vi "EmulationSandboxKeyboard.vi"() -> ()   [LabVIEW 2026]
uses:
  KeyboardAndMouseDataAcquisition.ctl
  replay/KeyboardReplayKey.ctl
  KeyType.ctl
  <vilib>/Wovalab/Utilities/Helper Loop Periodic Timing/Helper Loop Periodic Timing.lvclass/Helper Loop Periodic Timing.ctl
  MouseLUTSelector.ctl
  aee89bbf-916d-4481-9317-930c4b9b316a.vi
  be5614b6-9380-4e19-a85a-dfb08a87b78c.vi
  <vilib>/Wovalab/Utilities/Helper Loop Periodic Timing/Read Current Number Of Execution.vi
  <vilib>/Wovalab/Utilities/Helper Loop Periodic Timing/Stop Helper Loop Internal.vi
  <vilib>/Wovalab/Utilities/Helper Loop Periodic Timing/U32 Max Value--constant.vi
  <vilib>/Wovalab/Utilities/Helper Loop Periodic Timing/Update Last Execution Time.vi
  <vilib>/Wovalab/Utilities/Helper Loop Periodic Timing/Loops Events AE.vi
  <vilib>/Wovalab/Utilities/Helper Loop Periodic Timing/Notify Monitoring Window.vi
  <vilib>/Wovalab/Utilities/Helper Loop Periodic Timing/Monitoring--global.vi
  <userlib>/_OpenG.lib/comparison/comparison.llb/U8 Changed__ogtk.vi
  <vilib>/Wovalab/Utilities/Helper Loop Periodic Timing/Late Execution Mode--enum.ctl
  <vilib>/Wovalab/Utilities/Helper Loop Periodic Timing/Helper Loop Periodic Timing.lvclass
  replay/Replay/src/Libraries/Replay/Replay.lvlib
  <userlib>/_OpenG.lib/comparison/comparison.llb/openg_comparison__ogtk.lvlib
  a2901e3a-1446-44b0-a1b1-14ac9caae76d.vi
  User32.dll
panel:
  out "Array 4":T1(array[cluster])
  out "Array 2":T2(array[cluster])
  out "Array":T3(array[ring])
  out "Unimplemented":bool
  out "Boolean":bool
  out "error out":errorcluster
  out "ReplaySamples":T4[](array[typedef])
  in  "Run ID":string
  out "Virtual Key 2":T5=164
  in  "keyType Recorded":T6=enum."1"
  out "Virtual Key":T5=164
  out "Key":T7(ring)
  in  "Exit":bool
  in  "Stop":bool
  in  "Start":bool
  out "Keyboard Keys Pressed":T3(array[ring])
  out "Array 3":T4[](array[typedef])
  # "wqeeeeeeeeeeeeeeeeeeeeeeeeeeeeeeeeeeeeeeeeeeeeeeeeeeeeeeeeeeeeeeeeeeeeeeeeeeeeee"
  # "sssssssssssssddddddddddddddddddddddddddddddddddddddddddd"
  # "fsdsdsdsdsdsdsdsdsdsdaaaaaaaaaaaaaaaaaaaaaaaaaaaaaaaaa"
  # "qweeeeeeeeewqqqqqqqqqqqqqqqqqqqqqqqqqqqqqqqqqqqqqqqqqq"
  # "sdffffffffffffffffffAAAAAA"
  # "sdsdsdsdsdsdsdsdsdsdaaaaaaaaaaaaaaaaaaaaaaaaaaaaaaaaaaaaaaaaaaaaaaaaaaaaaaaaaaa"
  # "rewwwwwwwwwwwwwwwwwwwwrewwerrrrrrrrrewwwwwwwwwwwwww"
  # "rew"
  # "rrrrrrrrreeeeeeeewwwwwwwwww"
  # "rrrrrrrreeeeeeeeeeewwwwwwwwwwwwwww"
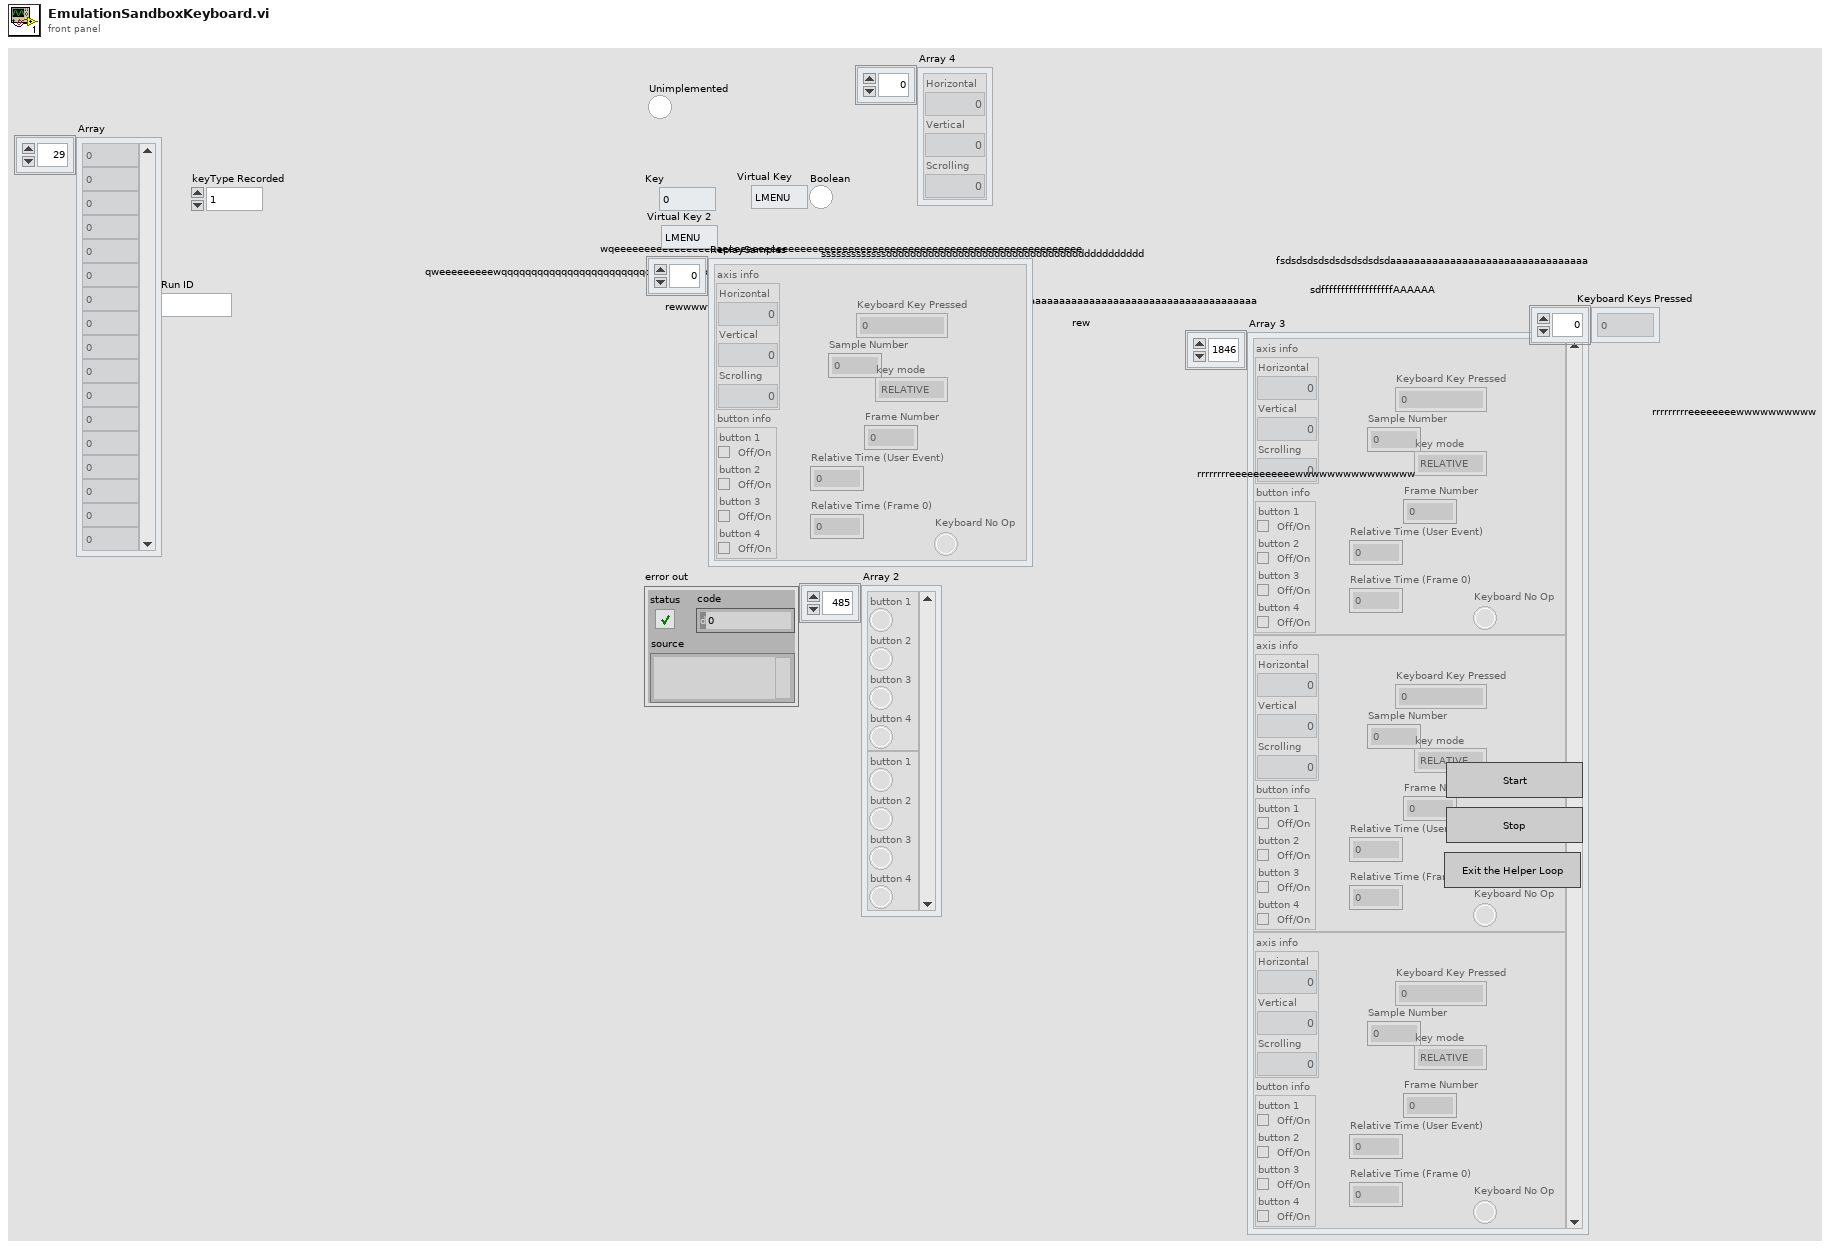
[diagram p1: front panel]
types:
  T1 = cluster{"Horizontal":i32, "Vertical":i32, "Scrolling":i32}[]
  T2 = cluster{"button 1":bool, "button 2":bool, "button 3":bool, "button 4":bool}[]
  T3 = enum16{"0", "1", "2", "3", "4", "5", "6", "7", "8", "9", "A", "B", "C", "D", "E", "F", "G", "H", "I", "J", "K", "L", "M", "N", "O", "P", "Q", "R", "S", "T", "U", "V", "W", "X", "Y", "Z", "F1", "F2", "F3", "F4", "F5", "F6", "F7", "F8", "F9", "F10", "F11", "F12", "F13", "F14", "F15", "ADD", "BACK", "BACKSLASH", "CAPITAL", "COMMA", "DECIMAL", "DELETE", "DIVIDE", "DOWN", "END", "EQUALS", "ESCAPE", "GRAVE (`)", "HOME", "INSERT", "LBRACKET", "LCONTROL", "LEFT", "L ALT", "LSHIFT", "LWIN", "MINUS", "MULTIPLY", "NEXT", "NUMLOCK", "NUMPAD_0", "NUMPAD_1", "NUMPAD_2", "NUMPAD_3", "NUMPAD_4", "NUMPAD_5", "NUMPAD_6", "NUMPAD_7", "NUMPAD_8", "NUMPAD_9", "PAUSE", "PERIOD", "PRIOR (PG UP)", "RBRACKET", "RCONTROL", "RETURN", "RIGHT", "R ALT", "RSHIFT", "RWIN", "SCROLL", "SEMICOLON", "SLASH", "SPACE", "SUBTRACT", "TAB", "UP", "ENTER (num pad)", "' (quote)"}[]
  T4 = typedef "KeyboardAndMouseDataAcquisition.ctl" = cluster{"axis info":cluster{"Horizontal":i32, "Vertical":i32, "Scrolling":i32}, "button info":cluster{"button 1":bool, "button 2":bool, "button 3":bool, "button 4":bool}, "Relative Time (User Event)":dbl, "Sample Number":u32, "Relative Time (Frame 0)":dbl, "key mode":enum16{"RELATIVE", "ABSOLUTE"}, "Frame Number":u32, "Keyboard Key Pressed":enum16{"0", "1", "2", "3", "4", "5", "6", "7", "8", "9", "A", "B", "C", "D", "E", "F", "G", "H", "I", "J", "K", "L", "M", "N", "O", "P", "Q", "R", "S", "T", "U", "V", "W", "X", "Y", "Z", "F1", "F2", "F3", "F4", "F5", "F6", "F7", "F8", "F9", "F10", "F11", "F12", "F13", "F14", "F15", "ADD", "BACK", "BACKSLASH", "CAPITAL", "COMMA", "DECIMAL", "DELETE", "DIVIDE", "DOWN", "END", "EQUALS", "ESCAPE", "GRAVE (`)", "HOME", "INSERT", "LBRACKET", "LCONTROL", "LEFT", "L ALT", "LSHIFT", "LWIN", "MINUS", "MULTIPLY", "NEXT", "NUMLOCK", "NUMPAD_0", "NUMPAD_1", "NUMPAD_2", "NUMPAD_3", "NUMPAD_4", "NUMPAD_5", "NUMPAD_6", "NUMPAD_7", "NUMPAD_8", "NUMPAD_9", "PAUSE", "PERIOD", "PRIOR (PG UP)", "RBRACKET", "RCONTROL", "RETURN", "RIGHT", "R ALT", "RSHIFT", "RWIN", "SCROLL", "SEMICOLON", "SLASH", "SPACE", "SUBTRACT", "TAB", "UP", "ENTER (num pad)", "' (quote)"}, "Keyboard No Op":bool}
  T5 = typedef "KeyboardReplayKey.ctl" = u8
  T6 = typedef "KeyType.ctl" = enum16{"0", "1", "2", "3", "4", "5", "6", "7", "8", "9", "A", "B", "C", "D", "E", "F", "G", "H", "I", "J", "K", "L", "M", "N", "O", "P", "Q", "R", "S", "T", "U", "V", "W", "X", "Y", "Z", "F1", "F2", "F3", "F4", "F5", "F6", "F7", "F8", "F9", "F10", "F11", "F12", "F13", "F14", "F15", "ADD", "BACK", "BACKSLASH", "CAPITAL", "COMMA", "DECIMAL", "DELETE", "DIVIDE", "DOWN", "END", "EQUALS", "ESCAPE", "GRAVE (`)", "HOME", "INSERT", "LBRACKET", "LCONTROL", "LEFT", "L ALT", "LSHIFT", "LWIN", "MINUS", "MULTIPLY", "NEXT", "NUMLOCK", "NUMPAD_0", "NUMPAD_1", "NUMPAD_2", "NUMPAD_3", "NUMPAD_4", "NUMPAD_5", "NUMPAD_6", "NUMPAD_7", "NUMPAD_8", "NUMPAD_9", "PAUSE", "PERIOD", "PRIOR (PG UP)", "RBRACKET", "RCONTROL", "RETURN", "RIGHT", "R ALT", "RSHIFT", "RWIN", "SCROLL", "SEMICOLON", "SLASH", "SPACE", "SUBTRACT", "TAB", "UP", "ENTER (num pad)", "' (quote)"}
  T7 = enum16{"0", "1", "2", "3", "4", "5", "6", "7", "8", "9", "A", "B", "C", "D", "E", "F", "G", "H", "I", "J", "K", "L", "M", "N", "O", "P", "Q", "R", "S", "T", "U", "V", "W", "X", "Y", "Z", "F1", "F2", "F3", "F4", "F5", "F6", "F7", "F8", "F9", "F10", "F11", "F12", "F13", "F14", "F15", "ADD", "BACK", "BACKSLASH", "CAPITAL", "COMMA", "DECIMAL", "DELETE", "DIVIDE", "DOWN", "END", "EQUALS", "ESCAPE", "GRAVE (`)", "HOME", "INSERT", "LBRACKET", "LCONTROL", "LEFT", "L ALT", "LSHIFT", "LWIN", "MINUS", "MULTIPLY", "NEXT", "NUMLOCK", "NUMPAD_0", "NUMPAD_1", "NUMPAD_2", "NUMPAD_3", "NUMPAD_4", "NUMPAD_5", "NUMPAD_6", "NUMPAD_7", "NUMPAD_8", "NUMPAD_9", "PAUSE", "PERIOD", "PRIOR (PG UP)", "RBRACKET", "RCONTROL", "RETURN", "RIGHT", "R ALT", "RSHIFT", "RWIN", "SCROLL", "SEMICOLON", "SLASH", "SPACE", "SUBTRACT", "TAB", "UP", "ENTER (num pad)", "' (quote)"}
  T8 = typedef "Wovalab_lib_Utilities.lvlib/Helper Loop Periodic Timing.lvclass/Late Execution Mode--enum.ctl" = enum16{"No change", "Process missed periods ignoring original phase", "Process missed periods maintaining original phase"}
  T9 = typedef "MouseLUTSelector.ctl" = enum16{"Initialize", "Get Button and Axis Info", "Assign Button and Axis Info to Sample Number"}
  T10 = typedef "SerializedKeyPress.ctl" = cluster{"Key Down":bool, "Key Up":bool, "Key":enum16{"0", "1", "2", "3", "4", "5", "6", "7", "8", "9", "A", "B", "C", "D", "E", "F", "G", "H", "I", "J", "K", "L", "M", "N", "O", "P", "Q", "R", "S", "T", "U", "V", "W", "X", "Y", "Z", "F1", "F2", "F3", "F4", "F5", "F6", "F7", "F8", "F9", "F10", "F11", "F12", "F13", "F14", "F15", "ADD", "BACK", "BACKSLASH", "CAPITAL", "COMMA", "DECIMAL", "DELETE", "DIVIDE", "DOWN", "END", "EQUALS", "ESCAPE", "GRAVE (`)", "HOME", "INSERT", "LBRACKET", "LCONTROL", "LEFT", "L ALT", "LSHIFT", "LWIN", "MINUS", "MULTIPLY", "NEXT", "NUMLOCK", "NUMPAD_0", "NUMPAD_1", "NUMPAD_2", "NUMPAD_3", "NUMPAD_4", "NUMPAD_5", "NUMPAD_6", "NUMPAD_7", "NUMPAD_8", "NUMPAD_9", "PAUSE", "PERIOD", "PRIOR (PG UP)", "RBRACKET", "RCONTROL", "RETURN", "RIGHT", "R ALT", "RSHIFT", "RWIN", "SCROLL", "SEMICOLON", "SLASH", "SPACE", "SUBTRACT", "TAB", "UP", "ENTER (num pad)", "' (quote)"}}
  T11 = cluster{"Horizontal":i32, "Vertical":i32, "Scrolling":i32}
  T12 = cluster{"button 1":bool, "button 2":bool, "button 3":bool, "button 4":bool}
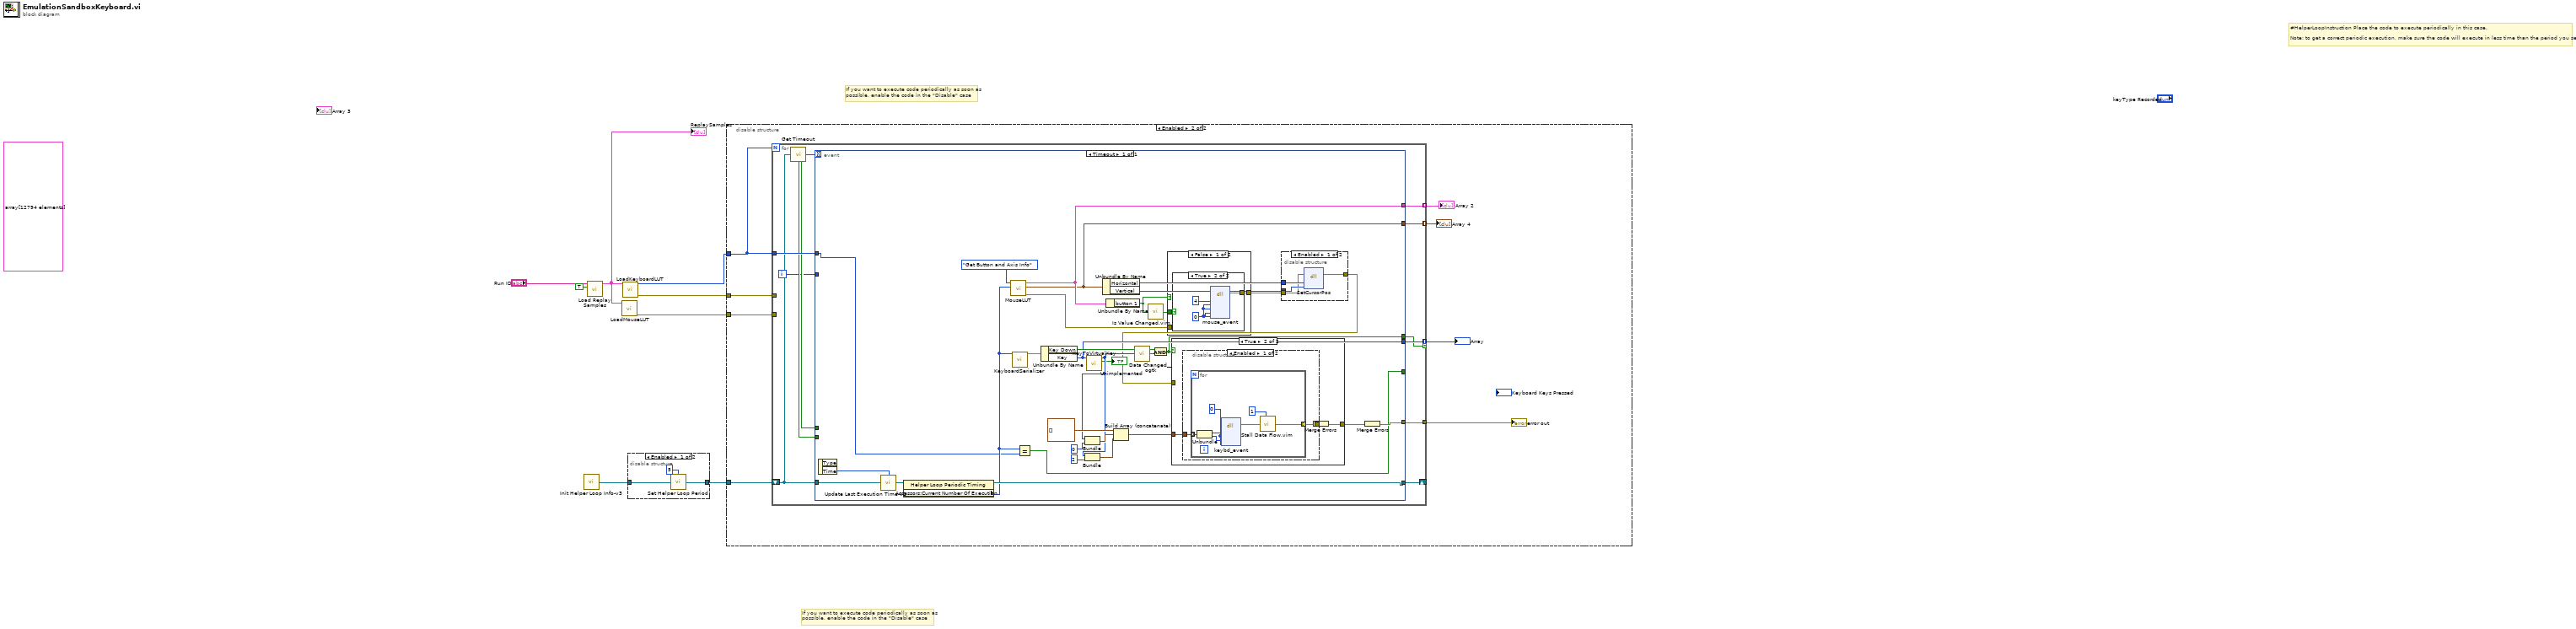
[diagram p0: block diagram]
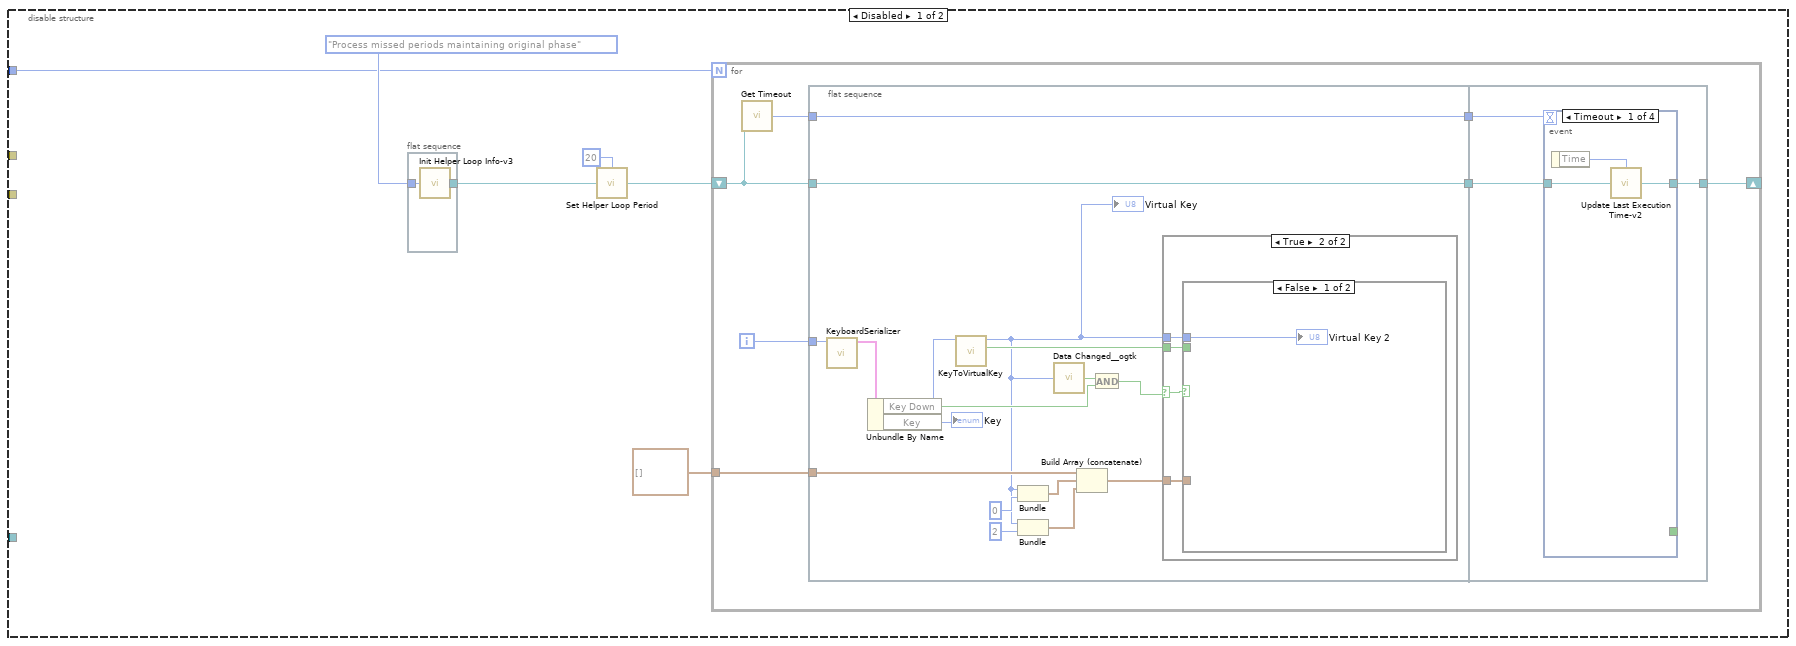
[diagram p3: hidden frame]
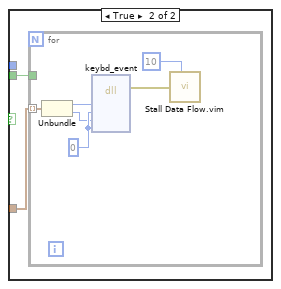
[diagram p5: hidden frame]
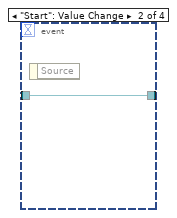
[diagram p6: hidden frame]
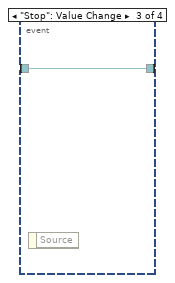
[diagram p7: hidden frame]
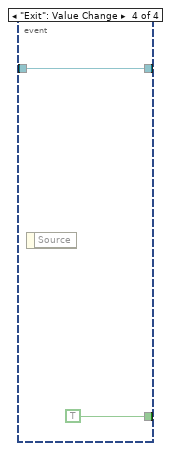
[diagram p8: hidden frame]
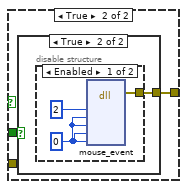
[diagram p11: hidden frame]
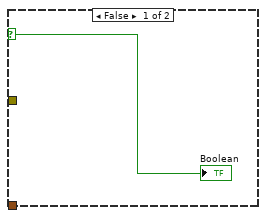
[diagram p14: hidden frame]
diagram:
  (unwired) T4[] array[12794 elements] ("Array 3")
  # "If you want to execute code periodically as soon as possible, enable the code in the \"Disable\" case"
  # "If you want to execute code periodically as soon as possible, enable the code in the \"Disable\" case"
  # "#HelperLoopInstruction Place the code to execute periodically in this case.\n\nNote: to get a correct periodic execution, make sure the code will execute in less time than the period you set."
  n1 = call <vilib>:"Init Helper Loop Info-v3.vi"() -> ("Helper Loop Periodic Timing"=w4:refnum<class "Helper Loop Periodic Timing.lvclass">)  [unwired: 2 in]
  n2 = call "Load Replay Samples.vi"("Load From ProgramData"=TRUE, "Run ID"="Run ID") -> ("ReplaySamples"=w2:T4[])  [unwired: 8 in, 1 out]
  "ReplaySamples" <- w2
  n3 = call "LoadMouseLUT.vi"("Metadata"=w2) -> ("error out"=w1:errorcluster)  [unwired: 10 in]
  n4 = call "LoadKeyboardLUT.vi"("Metadata"=w2) -> ("error out"=w6:errorcluster, "Samples"=w5:u32)  [unwired: 9 in]
  n5 = disable-structure shown="Enabled" {
    disable-tunnel: w4 -> [w11 w12]
    disable-tunnel: [w10 w12] -> w3
    frame Enabled {
      n6 = call <vilib>:"Set Helper Loop Period.vi"("Period (ms)"=5, "Helper Loop Periodic Timing in"=w11) -> ("Helper Loop Periodic Timing out"=w10:refnum<class "Helper Loop Periodic Timing.lvclass">)  [unwired: 13 in]
    }
    frame Disabled {
    }
  }
  n7 = disable-structure shown="Enabled" {
    disable-tunnel: w5 -> [w13 w75]
    disable-tunnel: w6 -> [_ w76]
    disable-tunnel: w3 -> [_ w74]
    disable-tunnel: w1 -> [_ w73]
    frame Disabled {
      n8 = flat-sequence {
        tunnel: [w69] -> w17
        tunnel: Late_Execution_Mode--enum."Process missed periods maintaining original phase" ("Late Execution Mode (Process missed periods ignoring original phase)") -> [w68]
        frame #0 {
          n9 = call <vilib>:"Init Helper Loop Info-v3.vi"("Late Execution Mode (Process missed periods ignoring original phase)"=w68) -> ("Helper Loop Periodic Timing"=w69:refnum<class "Helper Loop Periodic Timing.lvclass">)  [unwired: 1 in]
        }
      }
      n10 = call <vilib>:"Set Helper Loop Period.vi"("Period (ms)"=20, "Helper Loop Periodic Timing in"=w17) -> ("Helper Loop Periodic Timing out"=w18:refnum<class "Helper Loop Periodic Timing.lvclass">)  [unwired: 13 in]
      n11 = for {
        N: w13 -> [_]
        shift-right: [w23] -> _
        shift-left: w18 -> [w24]
        tunnel: cluster{i32, i32}[] [] -> [w20]
        i -> [w19]
        n12 = call <vilib>:"Get Timeout.vi"("Helper Loop Periodic Timing"=w24) -> ("Timeout (ms)"=w25:i32)  [unwired: 12 in, 2 out]
        n13 = flat-sequence {
          tunnel: w24 -> [w40]
          tunnel: w25 -> [w41]
          tunnel: [w41] -> w22
          tunnel: [w40] -> w21
          tunnel: w20 -> [w35]
          tunnel: w19 -> [w29]
          tunnel: [w55] -> w23
          tunnel: w22 -> [w57]
          tunnel: w21 -> [w56]
          frame #0 {
            n14 = call "KeyboardSerializer.vi"("Sample Number"=w29) -> ("SerializedKeyPress"=w28:T10)  [unwired: 9 in, 1 out]
            n15 = Unbundle By Name(w28) -> ("Key Down"=w31:bool, "Key"=w39:T7)
            "Key" <- w39
            n16 = call "KeyToVirtualKey.vi"("keyType Recorded"=w39) -> ("Unimplemented"=w27:bool, "Virtual Key"=w26:T5)  [unwired: 9 in]
            "Virtual Key" <- w26
            n17 = Bundle("Virtual Key"=w26, 0) -> (w37:cluster{"Virtual Key":T5, i32})  [unwired: 1 in]
            n18 = Bundle("Virtual Key"=w26, 2) -> (w38:cluster{"Virtual Key":T5, i32})  [unwired: 1 in]
            n19 = call-poly <userlib>:"Data Changed__ogtk.vi"("U8"=w26) -> ("Changed"=w32:bool)
            n20 = Build Array (concatenate)(w35, w37, w38) -> (w33:cluster{"Virtual Key":i32, i32}[])
            n21 = And(x=w32, y=w31) -> (x .and. y?=w30:bool)
            n22 = case shown="True" w30 {
              selector: w30 -> [_ w43]
              tunnel: w33 -> [_ w45]
              tunnel: w27 -> [_ w44]
              tunnel: w26 -> [_ w42]
              frame False {
              }
              frame True {
                n23 = case shown="False" w43 {
                  tunnel: w45 -> [_ w48]
                  tunnel: w44 -> [_ w47]
                  tunnel: w42 -> [w46 _]
                  frame False {
                    "Virtual Key 2" <- w46
                  }
                  frame True {
                    n24 = for {
                      tunnel: w48 -> [w53] mode=indexing
                      tunnel: w47 -> [_]
                      w54 = u32 0 ("dwFlags")
                      n25 = Unbundle(w53) -> ("Virtual Key"=w52:i32, w51:i32)
                      n26 = dll-call lib="user32.dll" fn="keybd_event"("bVk"=w52, "bScan"=w54, "dwFlags"=w51, "dwExtraInfo"=w54) -> (error out=w50:errorcluster)  [unwired: 8 in, 1 out]
                      n27 = call "Stall Data Flow.vim"("value in"=w50, "milliseconds to wait"=u32 10) -> ()  [unwired: 2 out]
                    }
                  }
                }
              }
            }
          }
          frame #1 {
            n28 = event shown="[0] Timeout" {
              selector: _ -> [_ _ _ _]
              dyn-events: _ -> [_ _ _ _]
              timeout: w57 -> [_ _ _ _]
              tunnel: w56 -> [w60 w63 w65 w67]
              tunnel: [w59 w62 w64 w67] -> w55
              tunnel: [_ _ _ TRUE] -> _
              event Timeout {
                n29 = event-data() -> ("Time"=w58:u32)  [unwired: 1 in]
                n30 = call <vilib>:"Update Last Execution Time-v2.vi"("Time"=w58, "Helper Loop Periodic Timing in"=w60) -> ("Helper Loop Periodic Timing out"=w59:refnum<class "Helper Loop Periodic Timing.lvclass">)  [unwired: 12 in, 1 out]
              }
              event "Start": Value Change {
                # "#HelperLoopInstruction Set the desired period (in ms), here."
                n31 = call <vilib>:"Set Helper Loop Period.vi"("Period (ms)"=500, "Helper Loop Periodic Timing in"=w63) -> ("Helper Loop Periodic Timing out"=w62:refnum<class "Helper Loop Periodic Timing.lvclass">)  [unwired: 13 in]
                n32 = event-data() -> ()  [unwired: 1 in, 1 out]
              }
              event "Stop": Value Change {
                n33 = call <vilib>:"Stop Helper Loop.vi"("Helper Loop Periodic Timing in"=w65) -> ("Helper Loop Periodic Timing out"=w64:refnum<class "Helper Loop Periodic Timing.lvclass">)
                n34 = event-data() -> ()  [unwired: 1 in, 1 out]
              }
              event "Exit": Value Change {
                n35 = event-data() -> ()  [unwired: 1 in, 1 out]
              }
            }
          }
        }
      }
    }
    frame Enabled {
      n36 = for {
        N: w75 -> [_]
        tunnel: [w89] -> w77
        tunnel: w76 -> [_]
        tunnel: w75 -> [w88]
        shift-right: [w83] -> _
        shift-left: w74 -> [w87]
        tunnel: w73 -> [_]
        tunnel: [w81] -> w72 mode=indexing if=w80
        tunnel: [w79] -> w71 mode=indexing
        tunnel: [w78] -> w70 mode=indexing
        i -> [w82]
        n37 = call <vilib>:"Get Timeout.vi"("Helper Loop Periodic Timing"=w87) -> ("Timeout (ms)"=w86:i32, "Late?"=w84:bool, "First Execution Since Period Modification?"=w85:bool)  [unwired: 12 in]
        n38 = event shown="[0] Timeout" {
          selector: _ -> [_]
          dyn-events: _ -> [_]
          timeout: w86 -> [_]
          tunnel: [w104] -> w89
          tunnel: w88 -> [w96]
          tunnel: w87 -> [w101]
          tunnel: w85 -> [_]
          tunnel: w84 -> [_]
          tunnel: [w98] -> w83
          tunnel: w82 -> [_]
          tunnel: [w95] -> _
          tunnel: [w94] -> w81
          tunnel: [w93] -> w80
          tunnel: [w92] -> w79
          tunnel: [w91] -> w78
          event Timeout {
            n39 = event-data() -> ("Time"=w100:u32)  [unwired: 1 in, 1 out]
            n40 = call <vilib>:"Update Last Execution Time-v2.vi"("Time"=w100, "Helper Loop Periodic Timing in"=w101) -> ("Helper Loop Periodic Timing out"=w99:refnum<class "Helper Loop Periodic Timing.lvclass">)  [unwired: 12 in, 1 out]
            n41 = property class="Helper Loop Periodic Timing"(reference=w99) -> (reference out=w98:refnum<class "Helper Loop Periodic Timing.lvclass">, "Accessors:Current Number Of Execution"=w97:u64)  [unwired: 1 in, 1 out]
            n42 = call "MouseLUT.vi"("Sample Number"=w97, "LUT Selector"=MouseLUTSelector."Get Button and Axis Info") -> ("error out"=w107:errorcluster, "axis info out"=w91:T11, "button info out"=w92:T12)  [unwired: 7 in]
            n43 = call "KeyboardSerializer.vi"("Sample Number"=w97) -> ("SerializedKeyPress"=w105:T10)  [unwired: 9 in, 1 out]
            n44 = Equal?(x=w97, y=w96) -> (x = y?=w95:bool)
            n45 = Unbundle By Name(w105) -> ("Key Down"=w112:bool, "Key"=w94:T7)
            n46 = call "KeyToVirtualKey.vi"("keyType Recorded"=w94) -> ("Unimplemented"=→"Unimplemented":bool, "Virtual Key"=w103:T5)  [unwired: 9 in]
            n47 = Bundle("Virtual Key"=w103, 0) -> (w117:cluster{"Virtual Key":T5, i32})  [unwired: 1 in]
            n48 = Bundle("Virtual Key"=w103, 2) -> (w118:cluster{"Virtual Key":T5, i32})  [unwired: 1 in]
            n49 = Unbundle By Name(w91) -> ("Horizontal"=w121:i32, "Vertical"=w120:i32)
            n50 = Unbundle By Name(w92) -> ("button 1"=w119:bool)
            n51 = Build Array (concatenate)(cluster{i32, i32}[] [], w117, w118) -> (w106:cluster{"Virtual Key":i32, i32}[])
            n52 = call-poly <userlib>:"Data Changed__ogtk.vi"("U8"=w103) -> ("Changed"=w113:bool)
            n53 = call "Is Value Changed.vim"("value"=w119) -> ("changed or first call?"=w110:bool)
            n54 = And(x=w112, y=w113) -> (x .and. y?=w93:bool)
            n55 = case shown="False" w119 {
              tunnel: w110 -> [w128 w133]
              tunnel: [w127 w132] -> w109
              tunnel: w107 -> [_ _]
              frame False {
                n56 = case shown="True" w128 {
                  tunnel: [_ w129] -> w127
                  frame False {
                  }
                  frame True {
                    w130 = u32 0 ("dy")
                    n57 = dll-call lib="user32.dll" fn="mouse_event"("dwFlags"=u32 4, "dx"=w130, "dy"=w130, "dwData"=w130, "dwExtraInfo"=w130) -> (error out=w129:errorcluster)  [unwired: 9 in, 1 out]
                  }
                }
              }
              frame True {
                n58 = case shown="True" w133 {
                  tunnel: [_ w134] -> w132
                  frame False {
                  }
                  frame True {
                    n59 = disable-structure shown="Enabled" {
                      disable-tunnel: [w135 _] -> w134
                      frame Enabled {
                        w136 = u32 0 ("dy")
                        n60 = dll-call lib="user32.dll" fn="mouse_event"("dwFlags"=u32 2, "dx"=w136, "dy"=w136, "dwData"=w136, "dwExtraInfo"=w136) -> (error out=w135:errorcluster)  [unwired: 9 in, 1 out]
                      }
                      frame Disabled {
                      }
                    }
                  }
                }
              }
            }
            n61 = disable-structure shown="Enabled" {
              disable-tunnel: w121 -> [w125 _]
              disable-tunnel: w120 -> [w124 _]
              disable-tunnel: w109 -> [w123 w126]
              disable-tunnel: [w122 w126] -> w90
              frame Enabled {
                n62 = dll-call lib="User32.dll" fn="SetCursorPos" label="SetCursorPos (User32.dll)"(error in=w123, w125, w124) -> (error out=w122:errorcluster)  [unwired: 4 in, 2 out]
              }
              frame Disabled {
              }
            }
            n63 = case shown="True" w93 {
              selector: w93 -> [w138 _]
              tunnel: w106 -> [_ w140]
              tunnel: [_ w139] -> w108
              tunnel: w90 -> [_ _]
              frame False {
                "Boolean" <- w138
              }
              frame True {
                n64 = disable-structure shown="Enabled" {
                  disable-tunnel: w140 -> [w143 _]
                  disable-tunnel: [w141 _] -> w139
                  frame Enabled {
                    n65 = for {
                      tunnel: w143 -> [w149] mode=indexing
                      tunnel: [w144] -> w142 mode=indexing
                      w150 = u32 0 ("dwFlags")
                      n66 = Unbundle(w149) -> ("Virtual Key"=w148:i32, w147:i32)
                      n67 = dll-call lib="user32.dll" fn="keybd_event"("bVk"=w148, "bScan"=w150, "dwFlags"=w147, "dwExtraInfo"=w150) -> (error out=w146:errorcluster)  [unwired: 8 in, 1 out]
                      n68 = call "Stall Data Flow.vim"("value in"=w146, "milliseconds to wait"=u32 1) -> ("value out"=w144:errorcluster)  [unwired: 1 out]
                    }
                    n69 = Merge Errors(w142) -> (w141:errorcluster)
                  }
                  frame Disabled {
                  }
                }
              }
            }
            n70 = Merge Errors(w108) -> (w104:errorcluster)
          }
        }
      }
      "error out" <- w77
      "Array" <- w72
      "Array 2" <- w71
      "Array 4" <- w70
    }
  }
